vi "sns scratchpad.vi"() -> ()   [LabVIEW 2015]
uses:
  Core/HTTP Request/Region.ctl
  Core/HTTP Request/AWS Credentials.ctl
  Topic/Topic.lvclass
  Subscription/Subscription.lvclass
  Core/HTTP Request/HTTP Request.lvclass
panel:
  in  "AWS Credentials":T1
  in  "Region":T2
  out "error out":errorcluster
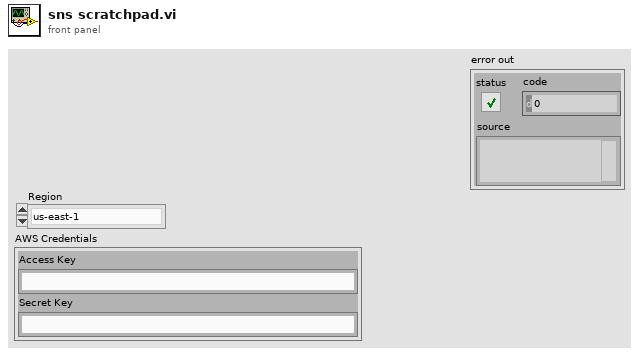
[diagram p1: front panel]
types:
  T1 = typedef "NI_AWS_Core.lvlib/HTTP Request.lvclass/AWS Credentials.ctl" = cluster{"Access Key":string, "Secret Key":string}
  T2 = typedef "NI_AWS_Core.lvlib/HTTP Request.lvclass/Region.ctl" = enum16{"us-east-1", "us-east-2", "us-west-1", "us-west-2", "ap-northeast-1", "ap-northeast-2", "ap-southeast-1", "ap-southeast-2", "ca-central-1", "eu-central-1", "eu-west-1", "eu-west-2", "sa-east-1"}
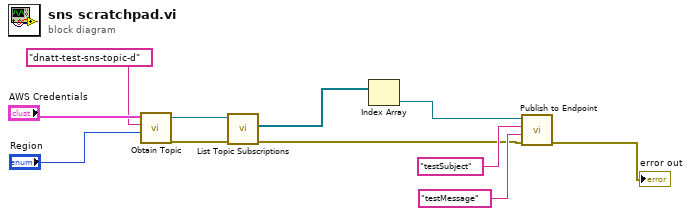
[diagram p0: block diagram]
diagram:
  n1 = call "Obtain Topic.vi"("Region"="Region", "Name"="dnatt-test-sns-topic-d", "AWS Credentials"="AWS Credentials") -> ("error out"=w4:errorcluster, "Topic out"=w5:refnum<class "Topic.lvclass">)  [unwired: 7 in]
  n2 = call "List Topic Subscriptions.vi"("error in (no error)"=w4, "Topic in"=w5) -> ("error out"=w3:errorcluster, "Subscriptions"=w2:refnum<class "Subscription.lvclass">[])  [unwired: 7 in, 1 out]
  n3 = Index Array(array=w2) -> (element=w1:refnum<class "Subscription.lvclass">)  [unwired: 1 in]
  n4 = call "Publish to Endpoint.vi"("error in (no error)"=w3, "Message"="testMessage", "Subject"="testSubject", "Subscription in"=w1) -> ("error out"=→"error out":errorcluster)  [unwired: 6 in, 1 out]
